vi "HOST_2518.vi"() -> ()   [LabVIEW 2018]
uses:
  <vilib>/userdefined/High Color/nirio_resource_hc.ctl
  <instrlib>/niDCPower/nidcpower.llb/niDCPower Measurement Type.ctl
  <vilib>/FPGAPlugInAG/PXI-7953R/niLvFpga_Open_PXI-7953R.vi
  <vilib>/rvi/interface/common/dynamic/niFpgaDynamicAddResources.vi
  <vilib>/FPGAPlugInAG/Dynamic/niLvFpga_Reset_Dynamic.vi
  <vilib>/FPGAPlugInAG/Dynamic/niLvFpga_Run_Dynamic.vi
  <vilib>/Utility/error.llb/Error Cluster From Error Code.vi
  <vilib>/rvi/errors/niLvFpgaAdjustHostInterfaceError.vi
  <vilib>/FPGAPlugInAG/Dynamic/niLvFpga_Close_Dynamic.vi
  <vilib>/rvi/interface/nirviOpenFPGA/nirviOpenFPGA.xnode
  FPGA Bitfiles/GMAX2518_FPGATarget_Target2518_wpKPnY-EnHw.lvbitx
  <vilib>/rvi/interface/nirviMethod/nirviMethod.xnode
  <vilib>/rvi/interface/nirviReadWriteControl/nirviReadWriteControl.xnode
  <vilib>/rvi/interface/nirviCloseFPGA/nirviCloseFPGA.xnode
  <vilib>/rvi/interface/Simulation/niFpgaSimulationCallBeginRW.vi
  <vilib>/FPGAPlugInAG/Dynamic/niLvFpga_ReadFifo_Dynamic.vi
  <vilib>/rvi/errors/niLvFpgaMergeErrorWithErrorCode.vi
  NiFpgaLv.dll
  <vilib>/FPGAPlugInAG/Dynamic/niLvFpga_StartFifo_Dynamic.vi
  <vilib>/FPGAPlugInAG/Dynamic/niLvFpga_WriteFifo_Dynamic.vi
panel:
  in  "Регистры":u8[](array[numeric])=[35, 5, 0, 100, 1, 0, 1, 0, 0, 0, 0, 0, 55, 16, 0, 0, 0, 69, 0, 6, 0, 160, 15, 0, 0, 0, 0, 0, 0, 0, 0, 0, 0, 0, 0, 0, 0, 0, 0, 0, 0, 0, 0, 0, 0, 0, 0, 0, 0, 0, 0, 0, 0, 0, 0, 0, 0, 0, 0, 0, 0, 0, 0, 0, 0, 0, 0, 0, 0, 0, 0, 0, 0, 0, 0, 0, 0, 0, 0, 0, 0, 0, 0, 52, 16, 0, 0, 6, 8, 2, 4, 0, 1, 33, 35, 2, 184, 100, 9, 50, 1, 160, 240, 255, 255, 255, 255, 255, 255, 255, 255, 255, 255, 255, 255, 2, 12, 80, 0, 25, 5, 76, 82, 65, 20, 3, 192, 96, 196, 71, 2, 12, 176, 3, 15, 48, 224, 240, 81, 72, 4, 192, 128, 196, 71, 62, 8, 1, 196, 255, 75, 164, 161, 64, 14, 65, 252, 31, 129, 12, 152, 0, 28, 28, 1, 8, 0, 0, 133, 2, 60, 64, 0, 18, 5, 224, 0, 196, 72, 1, 0, 3, 3, 48, 124, 20, 202, 68, 0, 0, 0, 0, 0, 0, 0, 0, 0, 0, 0, 0, 0, 0, 128, 0, 27, 33, 192, 83, 98, 60, 11, 16, 119, 196, 221, 13, 227, 143, 42, 0, 0, 0, 0, 0, 81, 0, 138, 162, 40, 40, 10, 138, 190, 31, 28, 1, 1, 0, 0, 40, 40, 40, 40, 232, 0, 0, 0, 0, 0, 0, 0, 0, 0, 0, 0, 0]
  out "Память":i32
  out "Image":T1(plugin-control)
  in  "12":u8=12
  in  "FR":u8=20
  in  "Хватит ждать!":bool
  out "Выкачали из памяти":bool
  out "SEU":u32
  in  "Upd_WR":bool
  out "FIFO_READ":i32
  in  "W(T)/R(F)":bool
  in  "Адрес":u8
  in  "Кол-во":u16=255
  out "НИ":bool
  out "READ":u8[](array[numeric])
  out "Прошили":bool
  in  "SPI":bool
  in  "Обнулить сбои":bool
  in  "Проверка сбоев":bool
  out "世男":bool
  in  "Период опроса, мс":u32=1
  in  "3,3V_LVDS, V":dbl=3.3 caption="voltage level" format="%_6p"
  in  "3,3V_LVDS_curlim":dbl=0.2 caption="current limit" format="%_6p"
  out "3,3V_LVDS_char":dbl(graph)=1.5967060684808935e-06
  in  "VDDPIX, V":dbl=3.6 caption="voltage level" format="%_6p"
  in  "VDDPIX_curlim":dbl=0.3 caption="current limit" format="%_6p"
  out "VDDPIX_char":dbl(graph)=1.5967060684808935e-06
  in  "VG_RSTH, V":dbl=4.1 caption="voltage level" format="%_6p"
  in  "VG_RSTH_curlim":dbl=0.1 caption="current limit" format="%_6p"
  out "VG_RSTH_char":dbl(graph)=1.5967060684808935e-06
  in  "LED, V":dbl=-8.0 caption="voltage level" format="%_6p"
  in  "LED_curlim":dbl=0.1 caption="current limit" format="%_6p"
  out "LED_char":dbl(graph)=1.5967060684808935e-06
  in  "VDD33A, V":dbl=3.3 caption="voltage level" format="%_6p"
  in  "VDD33A_curlim":dbl=0.3 caption="current limit" format="%_6p"
  out "VDD33A_char":dbl(graph)=1.5967060684808935e-06
  in  "VTXH, V":dbl=3.6 caption="voltage level" format="%_6p"
  in  "VDDIO, V":dbl=3.3 caption="voltage level" format="%_6p"
  in  "VDDCL, V":dbl=0.7 caption="voltage level" format="%_6p"
  in  "VDD13, V":dbl=1.3 caption="voltage level" format="%_6p"
  in  "VTXH_curlim":dbl=0.2 caption="current limit" format="%_6p"
  in  "VGRSTL_curlim":dbl=0.1 caption="current limit" format="%_6p"
  in  "VDDIO_curlim":dbl=0.1 caption="current limit" format="%_6p"
  in  "VDDCL_curlim":dbl=0.1 caption="current limit" format="%_6p"
  in  "VTXL_curlim":dbl=0.1 caption="current limit" format="%_6p"
  in  "VDD13_curlim":dbl=1.0 caption="current limit" format="%_6p"
  in  "VGRSTL, V":dbl=-1.3 caption="voltage level" format="%_6p"
  in  "VTXL, V":dbl=-1.3 caption="voltage level" format="%_6p"
  out "VTXH_char":dbl(graph)=-0.007753012065680951
  out "VGRSTL_char":dbl(graph)=6.909391540672134e-05
  out "VDDIO_char":dbl(graph)=9.424895165128459e-05
  out "VDDCL_char":dbl(graph)=-9.950040532110056e-06
  out "VTXL_char":dbl(graph)=9.067752968783287e-05
  out "VDD13_char":dbl(graph)=1.5967060684808935e-06
  in  "VDDPIX_selcur":dbl=0.2 caption="current limit" format="%_6p"
  in  "VDD33A_selcur":dbl=0.2 caption="current limit" format="%_6p"
  in  "VDD13_selcur":dbl=0.75 caption="current limit" format="%_6p"
  in  "VTXL_selcur":dbl=0.09 caption="current limit" format="%_6p"
  out "VDDCL_cur":dbl caption="measurement" format="%_6g"
  out "VTXL_cur":dbl caption="measurement" format="%_6g"
  out "VDD13_cur":dbl caption="measurement" format="%_6g"
  out "VDD33A_cur":dbl caption="measurement" format="%_6g"
  in  "SEL_Time, ms":u32=100
  in  "VG_RSTH_selcur":dbl=0.05 caption="current limit" format="%_6p"
  in  "VTXH_selcur":dbl=0.1 caption="current limit" format="%_6p"
  in  "VGRSTL_selcur":dbl=0.03 caption="current limit" format="%_6p"
  in  "VDDIO_selcur":dbl=0.03 caption="current limit" format="%_6p"
  in  "VDDCL_selcur":dbl=0.02 caption="current limit" format="%_6p"
  out "VDDPIX_cur":dbl caption="measurement" format="%_6g"
  out "VDDIO_cur":dbl caption="measurement" format="%_6g"
  out "VGRSTL_cur":dbl caption="measurement" format="%_6g"
  out "VTXH_cur":dbl caption="measurement" format="%_6g"
  out "VG_RSTH_cur":dbl caption="measurement" format="%_6g"
  out "VDDPIX":u16
  out "VDDPIX":bool
  out "VDD33A":u16
  out "VDD33A":bool
  out "VDD13":u16
  out "VDD13":bool
  out "VTXL":u16
  out "VTXL":bool
  in  "3":refnum<k15>="PXI1Slot5" caption="1"
  in  "MOVIE":bool
  in  "FRAME!":bool
  out "SEL":bool
  in  "SIM_SEL":bool
  out "VG_RSTH":u16
  out "VDDCL":u16
  out "VTXH":u16
  out "VDDIO":u16
  out "VGRSTL":u16
  out "VG_RSTH":bool
  out "VDDCL":bool
  out "VTXH":bool
  out "VDDIO":bool
  out "VGRSTL":bool
  in  "Стоп":bool
  in  "Питание":bool
  in  "LED":bool caption="output enabled"
  in  "0":refnum<k15>="PXI1Slot2" caption="1"
  in  "1":refnum<k15>="PXI1Slot3"
  in  "2":refnum<k15>="PXI1Slot4" caption="1"
  in  "resource name 2":T2="PXI1Slot6"
  in  "SEU":path=path "C:/LabView_PRJ/GMAX2518/SEU"
  in  "SEL":path=path "C:/LabView_PRJ/GMAX2518/SEL"
  out "Номер образца":string="1"
  # "0-163 тест (35)"
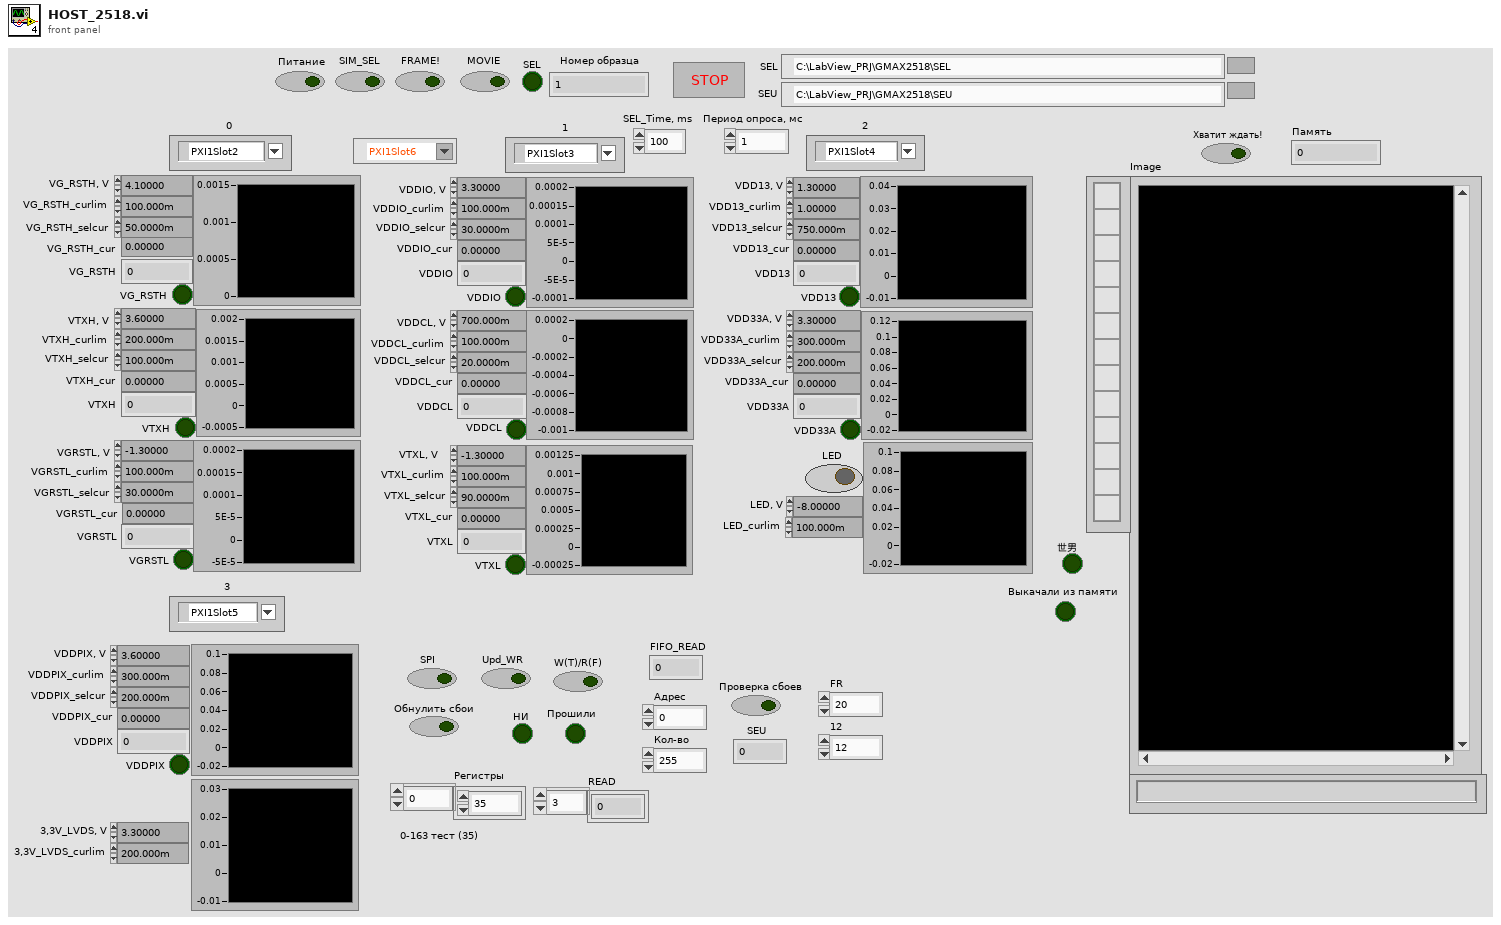
[diagram p1: front panel]
types:
  T1 = typedef "IMAQ Image.ctl" = refnum<image>
  T2 = typedef "nirio_resource_hc.ctl" = tag
  T3 = typedef "Image Type" = u32
  T4 = enum16{"open", "replace", "create", "open or create", "replace or create", "replace or create with confirmation"}
  T5 = typedef "niDCPower Measurement Type.ctl" = i32
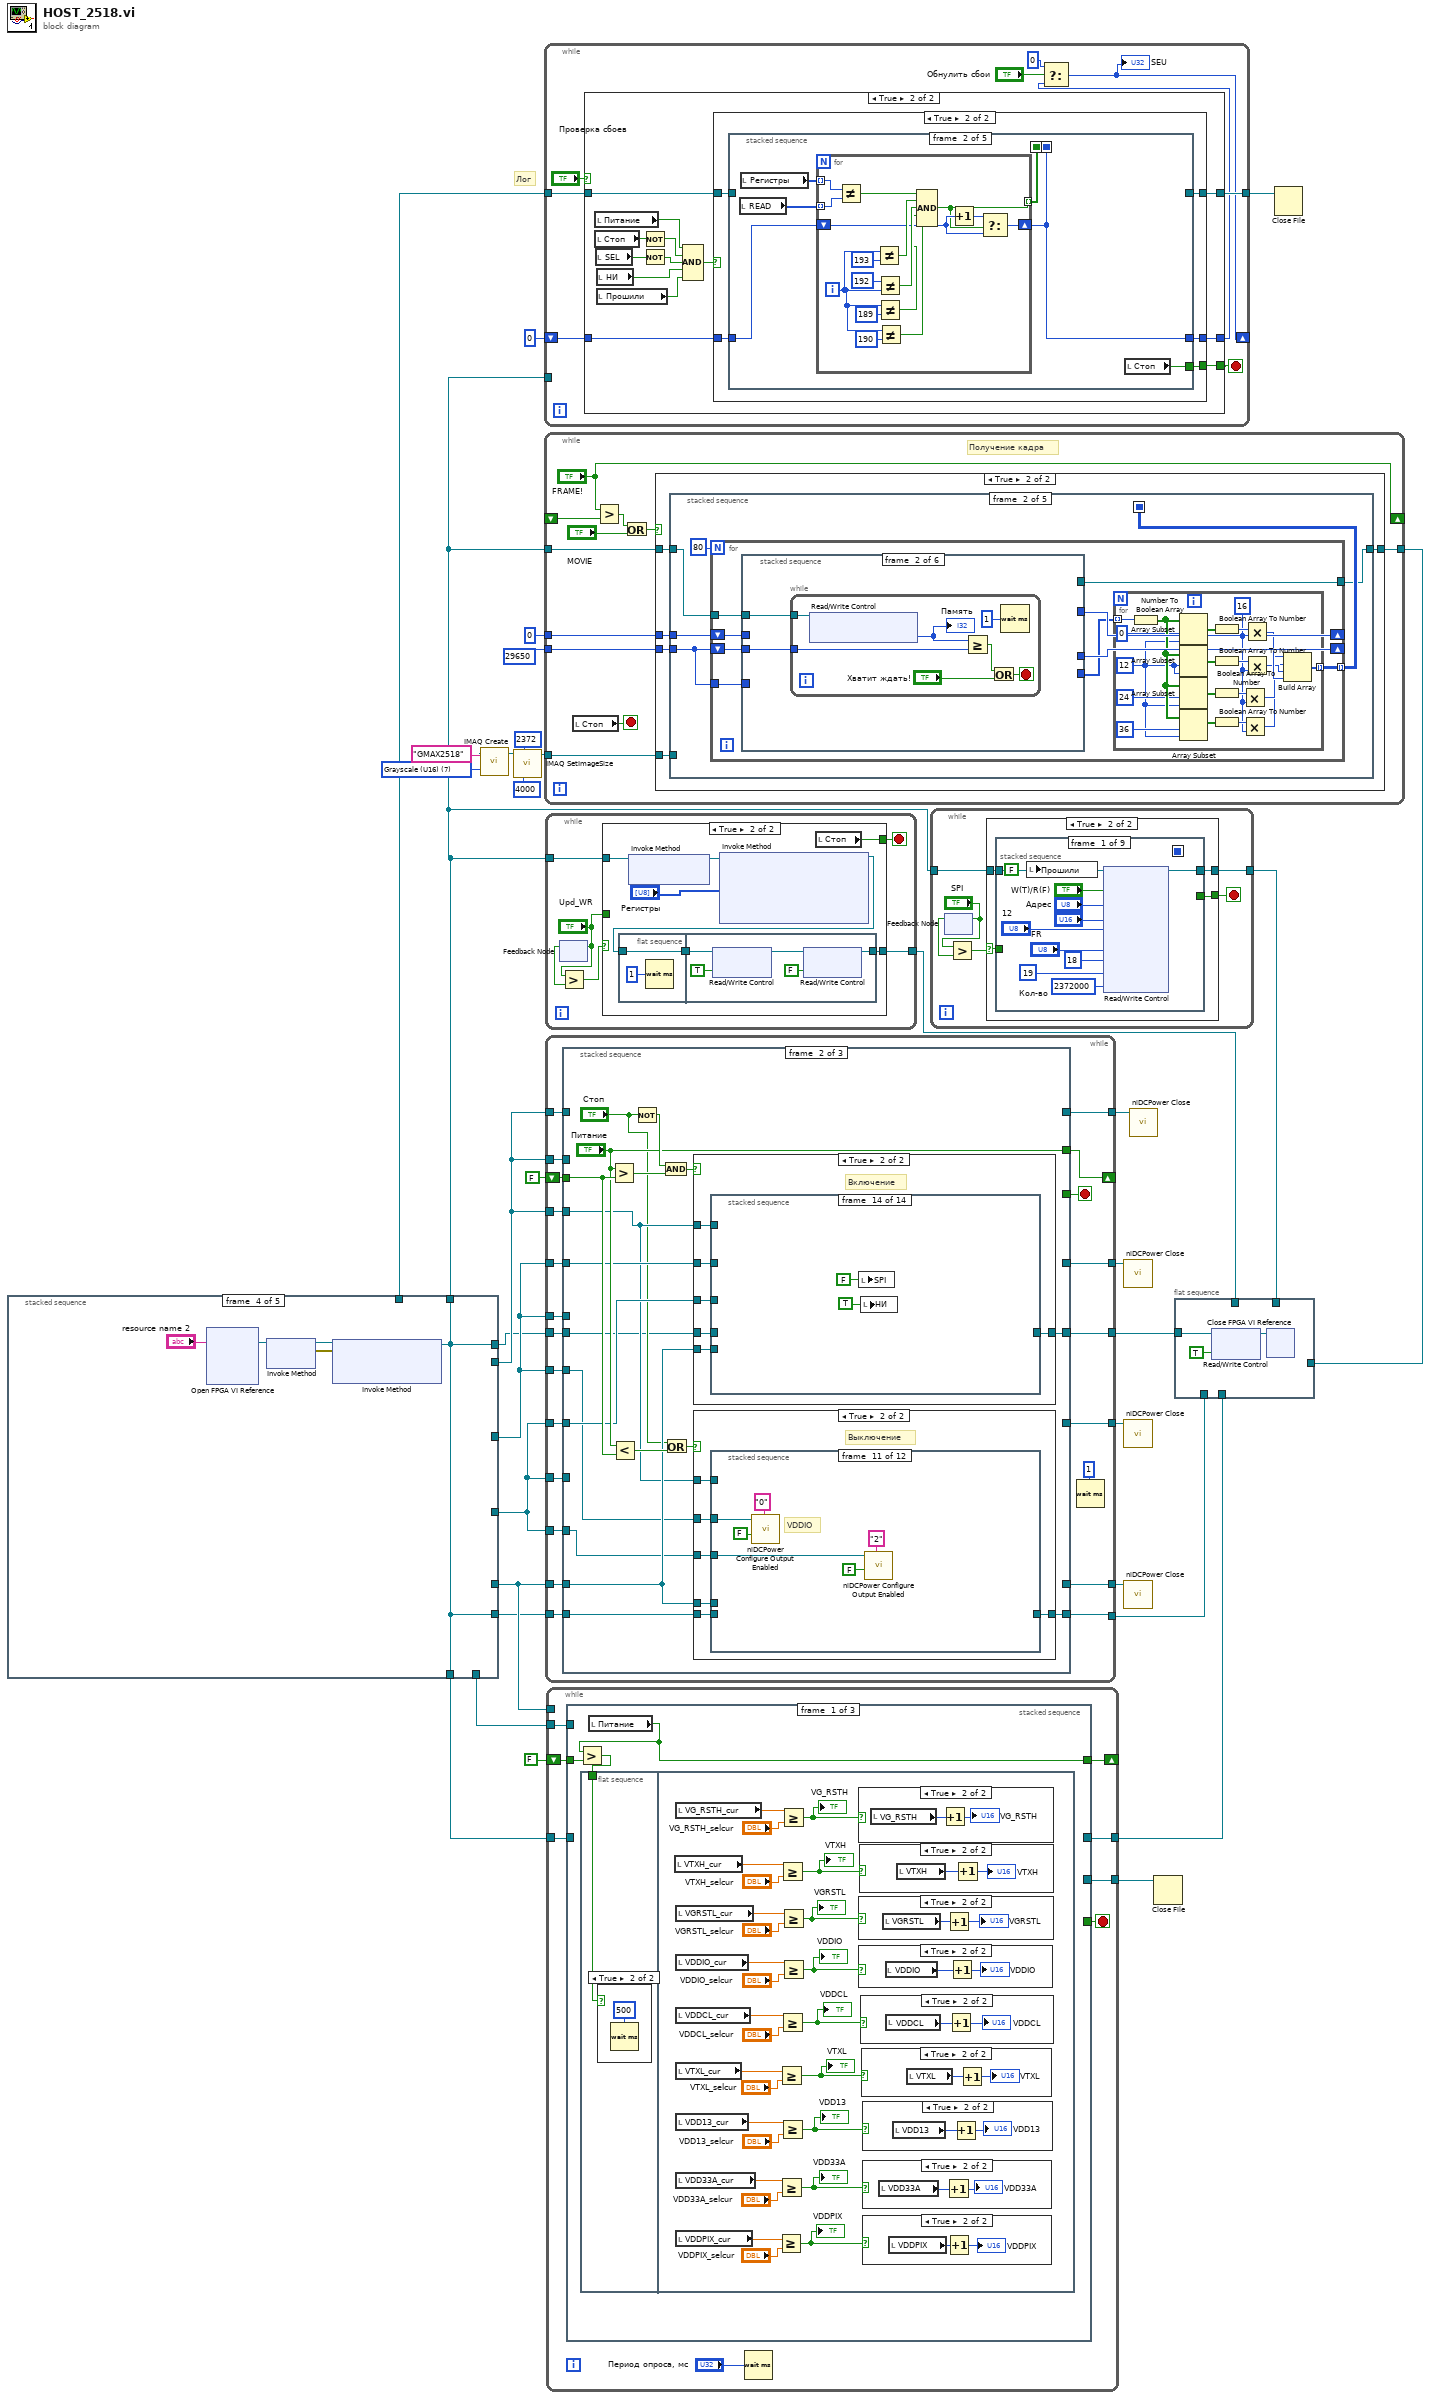
[diagram p0: block diagram]
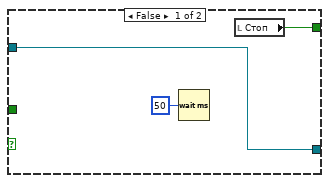
[diagram p2: hidden frame]
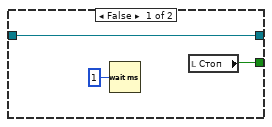
[diagram p3: hidden frame]
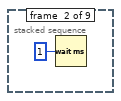
[diagram p4: hidden frame]
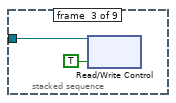
[diagram p5: hidden frame]
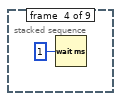
[diagram p6: hidden frame]
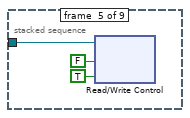
[diagram p7: hidden frame]
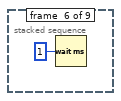
[diagram p8: hidden frame]
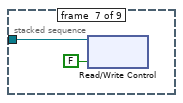
[diagram p9: hidden frame]
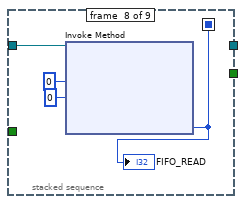
[diagram p10: hidden frame]
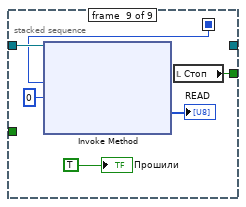
[diagram p11: hidden frame]
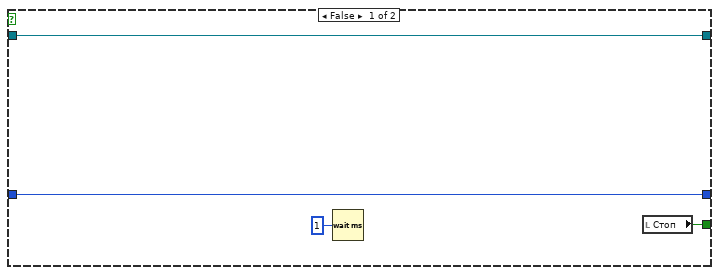
[diagram p12: hidden frame]
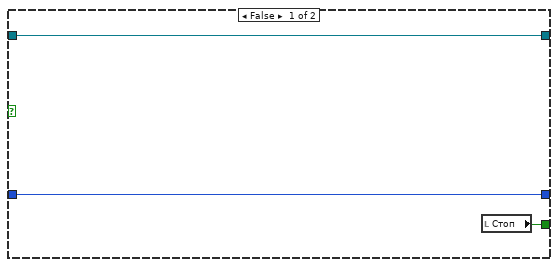
[diagram p13: hidden frame]
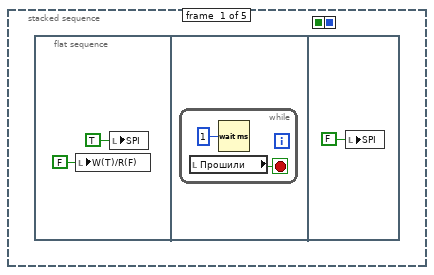
[diagram p14: hidden frame]
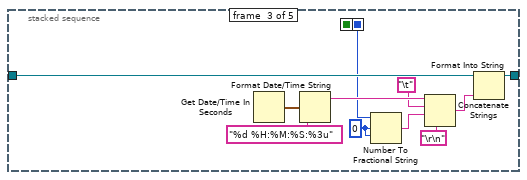
[diagram p15: hidden frame]
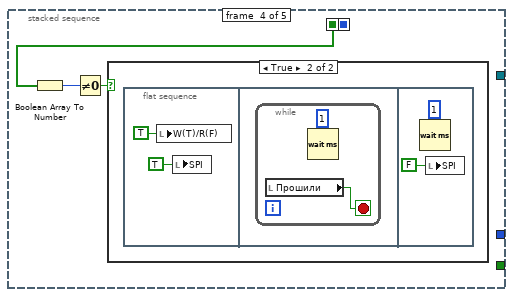
[diagram p16: hidden frame]
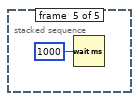
[diagram p18: hidden frame]
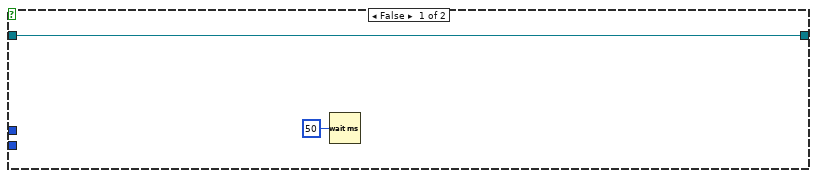
[diagram p19: hidden frame]
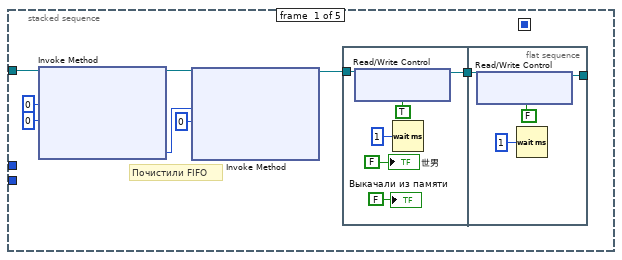
[diagram p20: hidden frame]
diagram:
  w20 = T3 7 items=["Grayscale (U8)", "Grayscale (I16)", "Grayscale (SGL)", "Complex (CSG)", "RGB (U32)", "HSL (U32)", "RGB (U64)", "Grayscale (U16)"] ("Image Type")
  # "Лог"
  n1 = stacked-sequence {
    tunnel: [_ _ _ _ w118] -> w26
    tunnel: [_ _ _ _ w111] -> w21
    tunnel: [_ _ _ _ w122] -> w27
    tunnel: [_ _ _ w106 _] -> w13
    tunnel: [_ _ _ w106 _] -> w30
    tunnel: [_ w45 _ _ _] -> w31
    tunnel: [_ _ _ w106 _] -> w12
    tunnel: [_ _ _ _ w112] -> w28
    tunnel: [_ _ w75 _ _] -> w1
    tunnel: [_ _ _ w106 _] -> w10
    frame #0 {
      w35 = FALSE ("Стоп")
      w34 = FALSE ("Стоп")
      w36 = u16 0 ("ADC")
      # "Обнуление"
      n2 = call "Begin.vi"() -> ("Номер образца 2"=→"Номер образца":string)  [unwired: 11 in]
      n3 = local write "VTXH"(w35) -> ()
      n4 = local write "SIM_SEL"(w35) -> ()
      n5 = local write "SEL"(w35) -> ()
      n6 = local write "VTXL"(w35) -> ()
      n7 = local write "VDD13"(w35) -> ()
      n8 = local write "VDD33A"(w35) -> ()
      n9 = local write "VDDPIX"(w35) -> ()
      n10 = local write "VTXH"(w36) -> ()
      n11 = local write "VDDCL"(w36) -> ()
      n12 = local write "VG_RSTH"(w36) -> ()
      n13 = local write "VDDIO"(w36) -> ()
      n14 = local write "VGRSTL"(w36) -> ()
      n15 = local write "VTXL"(w36) -> ()
      n16 = local write "VDD13"(w36) -> ()
      n17 = local write "VDD33A"(w36) -> ()
      n18 = local write "VDDPIX"(w36) -> ()
      n19 = local write "Стоп"(w34) -> ()
      n20 = local write "Питание"(w34) -> ()
      n21 = local write "FRAME!"(w34) -> ()
      n22 = local write "MOVIE"(w34) -> ()
      n23 = local write "LED"(w34) -> ()
      n24 = local write "VG_RSTH"(w34) -> ()
      n25 = local write "VDDCL"(w34) -> ()
      n26 = local write "VGRSTL"(w34) -> ()
      n27 = local write "VDDIO"(w34) -> ()
      n28 = local write "Выкачали из памяти"(w34) -> ()
    }
    frame #1 {
      w40 = "\t"
      # "Лог по токам"
      n29 = local read "Номер образца"() -> (w67:string)
      n30 = Build Path(base path="SEL", name or relative path=w67) -> (appended path=w64:path)
      n31 = Get Date/Time In Seconds() -> (seconds since 1Jan1904=w61:timestamp)
      n32 = call <vilib>:"Check if File or Folder Exists.vi"("path"=w64) -> ("file or folder exists?"=w65:bool, "dup path"=w66:path)  [unwired: 8 in, 1 out]
      n33 = Format Date/Time String(time format string (%c)="%d %H.%M.%S", seconds (now)=w61) -> (date/time string=w59:string)  [unwired: 1 in]
      n34 = case shown="False" w65 {
        tunnel: w66 -> [w73 w74]
        tunnel: [w72 w74] -> w39
        frame False {
          n35 = Create Folder(path (use dialog)=w73) -> (created path=w72:path)  [unwired: 2 in, 2 out]
        }
        frame True {
        }
      }
      n36 = Concatenate Strings(w59, ".xls" ("string")) -> (w58:string)
      n37 = Build Path(base path=w39, name or relative path=w58) -> (appended path=w60:path)
      n38 = Open/Create/Replace File(file path (use dialog)=w60, operation (0:open)=T4."open or create", access (0:read/write)=enum16{"read/write", "read-only", "write-only"}."read/write") -> (refnum out=w62:refnum<file>)  [unwired: 3 in, 2 out]
      n39 = case shown="True" TRUE {
        tunnel: w62 -> [w68 w71]
        tunnel: [w68 w69] -> w57
        frame False {
        }
        frame True {
          n40 = Set File Position(refnum=w71, from (0:start)=enum16{"start", "end", "current"}."end") -> (refnum out=w69:refnum<file>)  [unwired: 2 in, 1 out]
        }
      }
      n41 = Format Into String(initial string=w57, "Time" ("input 1"), w40, "VG_RSTH_cur", w40, "VTXH_cur", w40, "VGRSTL_cur", w40, "VDDIO_cur", w40, "VDDCL_cur", w40, "VTXL_cur", w40, "VDD13_cur", w40, "VDD33A_cur", w40, "VDDPIX_cur", w40, "\r\n") -> (resulting string=w45:refnum<file>)  [unwired: 2 in, 1 out]
    }
    frame #2 {
      w78 = "\t"
      # "Лог по сбоям"
      n42 = local read "Номер образца"() -> (w82:string)
      n43 = Build Path(base path="SEU", name or relative path=w82) -> (appended path=w96:path)
      n44 = Get Date/Time In Seconds() -> (seconds since 1Jan1904=w94:timestamp)
      n45 = call <vilib>:"Check if File or Folder Exists.vi"("path"=w96) -> ("file or folder exists?"=w97:bool, "dup path"=w98:path)  [unwired: 8 in, 1 out]
      n46 = Format Date/Time String(time format string (%c)="%d %H.%M.%S", seconds (now)=w94) -> (date/time string=w92:string)  [unwired: 1 in]
      n47 = case shown="False" w97 {
        tunnel: w98 -> [w104 w105]
        tunnel: [w103 w105] -> w83
        frame False {
          n48 = Create Folder(path (use dialog)=w104) -> (created path=w103:path)  [unwired: 2 in, 2 out]
        }
        frame True {
        }
      }
      n49 = Concatenate Strings(w92, ".xls" ("string")) -> (w91:string)
      n50 = Build Path(base path=w83, name or relative path=w91) -> (appended path=w93:path)
      n51 = Open/Create/Replace File(file path (use dialog)=w93, operation (0:open)=T4."open or create", access (0:read/write)=enum16{"read/write", "read-only", "write-only"}."read/write") -> (refnum out=w95:refnum<file>)  [unwired: 3 in, 2 out]
      n52 = case shown="True" TRUE {
        tunnel: w95 -> [w99 w102]
        tunnel: [w99 w100] -> w90
        frame False {
        }
        frame True {
          n53 = Set File Position(refnum=w102, from (0:start)=enum16{"start", "end", "current"}."end") -> (refnum out=w100:refnum<file>)  [unwired: 2 in, 1 out]
        }
      }
      n54 = Format Into String(initial string=w90, "Time" ("input 1"), w78, "Регистр №" ("input 3"), w78, "Содержание" ("input 4"), w78, "Кол-во сбоев" ("input 7"), "\r\n") -> (resulting string=w75:refnum<file>)  [unwired: 2 in, 1 out]
    }
    frame #3 {
      n55 = xnode "Open FPGA VI Reference"("resource name"="resource name 2") -> ("FPGA VI Reference Out"=w107:refnum<k20>)  [unwired: 1 in, 1 out]
      n56 = xnode "Invoke Method"("FPGA VI Reference In"=w107) -> ("FPGA VI Reference Out"=w110:refnum<k20>, "error out"=w109:errorcluster)  [unwired: 1 in]
      n57 = xnode "Invoke Method"("FPGA VI Reference In"=w110, "error in"=w109) -> ("FPGA VI Reference Out"=w106:refnum<k20>)  [unwired: 1 in, 1 out]
    }
    frame #4 {
      n58 = call <instrlib>:"niDCPower Initialize.vi"("resource name"="2") -> ("error out"=w128:errorcluster, "instrument handle out"=w125:refnum<k15>)  [unwired: 3 in, 6 out]
      n59 = call <instrlib>:"niDCPower Initialize.vi"("resource name"="1") -> ("error out"=w126:errorcluster, "instrument handle out"=w123:refnum<k15>)  [unwired: 3 in, 6 out]
      n60 = call <instrlib>:"niDCPower Initialize.vi"("resource name"="3") -> ("error out"=w116:errorcluster, "instrument handle out"=w117:refnum<k15>)  [unwired: 3 in, 6 out]
      n61 = call <instrlib>:"niDCPower Initialize.vi"("resource name"="0") -> ("error out"=w127:errorcluster, "instrument handle out"=w124:refnum<k15>)  [unwired: 3 in, 6 out]
      n62 = call <instrlib>:"niDCPower Configure Voltage Level.vi"("error in (no error)"=w128, "voltage level"=0.0, "channel name"="0,1,2", "instrument handle"=w125) -> ("instrument handle out"=w118:refnum<k15>)  [unwired: 6 in, 1 out]
      n63 = call <instrlib>:"niDCPower Configure Voltage Level.vi"("error in (no error)"=w126, "voltage level"=0.0, "channel name"="0,1,2", "instrument handle"=w123) -> ("instrument handle out"=w122:refnum<k15>)  [unwired: 6 in, 1 out]
      n64 = call <instrlib>:"niDCPower Configure Voltage Level.vi"("error in (no error)"=w116, "voltage level"=0.0, "channel name"="0,1", "instrument handle"=w117) -> ("instrument handle out"=w112:refnum<k15>)  [unwired: 6 in, 1 out]
      n65 = call <instrlib>:"niDCPower Configure Voltage Level.vi"("error in (no error)"=w127, "voltage level"=0.0, "channel name"="0,1,2", "instrument handle"=w124) -> ("instrument handle out"=w111:refnum<k15>)  [unwired: 6 in, 1 out]
    }
  }
  n66 = call "IMAQ Create"("Image Name"="GMAX2518", "Image Type"=w20) -> ("New Image"=w3:T1)  [unwired: 3 in, 1 out]
  n67 = call "IMAQ SetImageSize"("Y Resolution"=4000, "X Resolution"=2372, "Image"=w3) -> ("Image Out"=w6:T1)  [unwired: 2 in, 1 out]
  n68 = while {
    tunnel: w1 -> [w143]
    tunnel: [w142] -> w14
    shift-right: [w135] -> _
    shift-left: u32 0 -> [w139]
    tunnel: w13 -> [_]
    stop <- w140 stop-if-true
    n69 = case shown="True" "Проверка сбоев" {
      tunnel: [w145 w153] -> w140
      tunnel: w143 -> [w146 w154]
      tunnel: [w146 w150] -> w142
      tunnel: w139 -> [w144 w152]
      tunnel: [w144 w151] -> w138
      frame False {
        n70 = Wait (ms)(milliseconds to wait=u32 1) -> ()  [unwired: 1 out]
        n71 = local read "Стоп"() -> (w145:bool)
      }
      frame True {
        n72 = local read "Питание"() -> (w159:bool)
        n73 = local read "Стоп"() -> (w160:bool)
        n74 = local read "SEL"() -> (w149:bool)
        n75 = local read "НИ"() -> (w156:bool)
        n76 = local read "Прошили"() -> (w148:bool)
        n77 = Not(x=w160) -> (.not. x?=w158:bool)
        n78 = Not(x=w149) -> (.not. x?=w157:bool)
        n79 = Compound Arithmetic op=AND(w159, w158, w157, w156, w148) -> (w155:bool)
        n80 = case shown="True" w155 {
          tunnel: w154 -> [w161 w168]
          tunnel: [w163 w167] -> w153
          tunnel: w152 -> [w162 w166]
          tunnel: [w162 w165] -> w151
          tunnel: [w161 w164] -> w150
          frame False {
            n81 = local read "Стоп"() -> (w163:bool)
          }
          frame True {
            n82 = stacked-sequence {
              seq-local: [_ w175 _ _ _] -> [_ _ w200 _ _]
              seq-local: [_ w174 _ _ _] -> [_ _ _ w207 _]
              tunnel: w168 -> [_ _ w205 _ _]
              tunnel: [_ w179 _ _ _] -> w167
              tunnel: w166 -> [_ w176 _ _ _]
              tunnel: [_ w175 _ _ _] -> w165
              tunnel: [_ _ w196 _ _] -> w164
              frame #0 {
                n83 = flat-sequence {
                  frame #0 {
                    n84 = local write "W(T)/R(F)"(FALSE ("W(T)/R(F)")) -> ()
                    n85 = local write "SPI"(TRUE ("SPI")) -> ()
                  }
                  frame #1 {
                    n86 = while {
                      stop <- w172 stop-if-true
                      n87 = local read "Прошили"() -> (w172:bool)
                      n88 = Wait (ms)(milliseconds to wait=u32 1) -> ()  [unwired: 1 out]
                    }
                  }
                  frame #2 {
                    n89 = local write "SPI"(FALSE ("SPI")) -> ()
                  }
                }
              }
              frame #1 {
                n90 = local read "READ"() -> (w178:u8[])
                n91 = local read "Регистры"() -> (w177:u8[])
                n92 = for {
                  tunnel: w178 -> [w189] mode=indexing
                  tunnel: w177 -> [w195] mode=indexing
                  shift-right: [w186] -> w175
                  shift-left: w176 -> [w187]
                  tunnel: [w185] -> w174 mode=indexing
                  i -> [w184]
                  n93 = Not Equal?(x=w195, y=w189) -> (x != y?=w192:bool)
                  n94 = Not Equal?(x=w184, y=193) -> (x != y?=w191:bool)
                  n95 = Not Equal?(x=192, y=w184) -> (x != y?=w190:bool)
                  n96 = Not Equal?(x=w184, y=189) -> (x != y?=w183:bool)
                  n97 = Not Equal?(x=w184, y=190) -> (x != y?=w182:bool)
                  n98 = Compound Arithmetic op=AND(w192, w191, w190, w183, w182) -> (w185:bool)
                  n99 = Increment(x=w187) -> (x+1=w188:u32)
                  n100 = Select(t=w188, s=w185, f=w187) -> (s? t:f=w186:u32)
                }
                n101 = local read "Стоп"() -> (w179:bool)
              }
              frame #2 {
                w199 = i16 0 ("width (-)")
                n102 = Get Date/Time In Seconds() -> (seconds since 1Jan1904=w204:timestamp)
                n103 = Format Date/Time String(time format string (%c)="%d %H:%M:%S:%3u", seconds (now)=w204) -> (date/time string=w202:string)  [unwired: 1 in]
                n104 = Number To Fractional String(number=w200, width (-)=w199, precision (6)=w199) -> (F-format string=w198:string)  [unwired: 1 in]
                n105 = Concatenate Strings(w202, "\t", w198, "\r\n") -> (w206:string)
                n106 = Format Into String(initial string=w205, w206) -> (resulting string=w196:refnum<file>)  [unwired: 2 in, 1 out]
              }
              frame #3 {
                n107 = Boolean Array To Number(Boolean array=w207) -> (number=w209:u32)
                n108 = Not Equal To 0?(x=w209) -> (x != 0?=w208:bool)
                n109 = case shown="True" w208 {
                  frame False {
                  }
                  frame True {
                    n110 = flat-sequence {
                      frame #0 {
                        n111 = local write "W(T)/R(F)"(TRUE ("W(T)/R(F)")) -> ()
                        n112 = local write "SPI"(TRUE ("SPI")) -> ()
                      }
                      frame #1 {
                        n113 = while {
                          stop <- w213 stop-if-true
                          n114 = local read "Прошили"() -> (w213:bool)
                          n115 = Wait (ms)(milliseconds to wait=u32 1) -> ()  [unwired: 1 out]
                        }
                      }
                      frame #2 {
                        n116 = Wait (ms)(milliseconds to wait=u32 1) -> ()  [unwired: 1 out]
                        n117 = local write "SPI"(FALSE ("SPI")) -> ()
                      }
                    }
                  }
                }
              }
              frame #4 {
                n118 = Wait (ms)(milliseconds to wait=u32 1000) -> ()  [unwired: 1 out]
              }
            }
          }
        }
      }
    }
    n119 = Select(t=u32 0, s="Обнулить сбои", f=w138) -> (s? t:f=w135:u32)
    "SEU" <- w135
  }
  n120 = while {
    tunnel: w13 -> [w224]
    shift-right: ["FRAME!"] -> _
    shift-left: _ -> [w227]
    tunnel: u32 0 -> [w223]
    tunnel: u32 29650 ("163840") -> [w222]
    tunnel: w6 -> [w218]
    tunnel: [w217] -> w2
    stop <- w221 stop-if-true
    # "Получение кадра"
    n121 = local read "Стоп"() -> (w221:bool)
    n122 = Greater?(x="FRAME!", y=w227) -> (0:w226:bool)
    n123 = Or(x=w226, y="MOVIE") -> (x .or. y?=w225:bool)
    n124 = case shown="True" w225 {
      tunnel: w224 -> [w228 w234]
      tunnel: w223 -> [_ w233]
      tunnel: w222 -> [_ w232]
      tunnel: w218 -> [_ w231]
      tunnel: [w228 w230] -> w217
      frame False {
        n125 = Wait (ms)(milliseconds to wait=u32 50) -> ()  [unwired: 1 out]
      }
      frame True {
        n126 = stacked-sequence {
          seq-local: [_ w254 _ _ _] -> [_ _ _ w322 _]
          tunnel: w234 -> [w238 w255 _ _ w336]
          tunnel: w233 -> [_ w257 _ _ _]
          tunnel: w232 -> [_ w256 _ _ _]
          tunnel: w231 -> [_ _ _ w329 _]
          tunnel: [_ w253 _ _ _] -> w230
          frame #0 {
            # "Почистили FIFO"
            n127 = xnode "Invoke Method"("FPGA VI Reference In"=w238, "Number of Elements"=u32 0, "Timeout (ms)"=0) -> ("FPGA VI Reference Out"=w237:refnum<k20>, "Elements Remaining"=w239:u32)  [unwired: 1 in, 2 out]
            n128 = xnode "Invoke Method"("FPGA VI Reference In"=w237, "Number of Elements"=w239, "Timeout (ms)"=0) -> ("FPGA VI Reference Out"=w236:refnum<k20>)  [unwired: 1 in, 3 out]
            n129 = flat-sequence {
              tunnel: w236 -> [w248]
              tunnel: [w244] -> w235
              tunnel: [w250] -> _
              tunnel: w235 -> [w249]
              frame #0 {
                n130 = xnode "Read/Write Control"("FPGA VI Reference In"=w248, "Кадр в память"=TRUE ("EXPOSURE")) -> ("FPGA VI Reference Out"=w244:refnum<k20>)  [unwired: 1 in, 1 out]
                n131 = Wait (ms)(milliseconds to wait=u32 1) -> ()  [unwired: 1 out]
                "世男" <- FALSE
                "Выкачали из памяти" <- FALSE ("Выкачали из памяти")
              }
              frame #1 {
                n132 = xnode "Read/Write Control"("FPGA VI Reference In"=w249, "Кадр в память"=FALSE) -> ("FPGA VI Reference Out"=w250:refnum<k20>)  [unwired: 1 in, 1 out]
                n133 = Wait (ms)(milliseconds to wait=u32 1) -> ()  [unwired: 1 out]
              }
            }
          }
          frame #1 {
            n134 = for {
              N: 80 -> [_]
              tunnel: w255 -> [w267]
              shift-right: [w264] -> _
              shift-left: w257 -> [w266]
              shift-right: [w263] -> _
              shift-left: w256 -> [w265]
              tunnel: w256 -> [w262]
              tunnel: [w260] -> w254 mode=indexing
              tunnel: [w259] -> w253
              n135 = stacked-sequence {
                tunnel: w267 -> [w293 w294 w303 w305 w307 w313]
                tunnel: w266 -> [w292 _ _ _ _ _]
                tunnel: w265 -> [w291 w295 _ _ _ _]
                tunnel: [w290 _ _ _ _ _] -> w264
                tunnel: [w289 _ _ _ _ _] -> w263
                tunnel: [_ _ _ _ _ w315] -> w261
                tunnel: [_ _ _ _ _ w314] -> w259
                tunnel: w262 -> [w288 _ _ _ _ _]
                frame #0 {
                  n136 = xnode "Read/Write Control"("FPGA VI Reference In"=w293, "Нач_адр"=w292, "Кон_адр"=w291) -> ()  [unwired: 1 in, 2 out]
                  n137 = Add(x=w292, y=w288) -> (x+y=w290:u32)
                  n138 = Add(x=w288, y=w291) -> (x+y=w289:u32)
                }
                frame #1 {
                  n139 = while {
                    tunnel: w295 -> [w300]
                    tunnel: w294 -> [w298]
                    stop <- w299 stop-if-true
                    n140 = xnode "Read/Write Control"("FPGA VI Reference In"=w298) -> ("Записали адресов"=w296:u32)  [unwired: 1 in, 2 out]
                    "Память" <- w296
                    n141 = Greater Or Equal?(x=w296, y=w300) -> (x >= y?=w302:bool)
                    n142 = Or(x=w302, y="Хватит ждать!") -> (x .or. y?=w299:bool)
                    n143 = Wait (ms)(milliseconds to wait=u32 1) -> ()  [unwired: 1 out]
                  }
                }
                frame #2 {
                  n144 = xnode "Read/Write Control"("FPGA VI Reference In"=w303, "Кадр на ПК"=TRUE ("HOST")) -> ()  [unwired: 1 in, 2 out]
                }
                frame #3 {
                  n145 = xnode "Read/Write Control"("FPGA VI Reference In"=w305, "Кадр на ПК"=FALSE ("HOST")) -> ()  [unwired: 1 in, 2 out]
                }
                frame #4 {
                  n146 = while {
                    tunnel: w307 -> [w309]
                    stop <- w310 stop-if-true
                    # "Записан FIFO?"
                    n147 = local read "Хватит ждать!"() -> (w308:bool)
                    n148 = xnode "Read/Write Control"("FPGA VI Reference In"=w309) -> ("Записали FIFO"=w311:bool)  [unwired: 1 in, 2 out]
                    n149 = Or(x=w311, y=w308) -> (x .or. y?=w310:bool)
                    n150 = Wait (ms)(milliseconds to wait=u32 1) -> ()  [unwired: 1 out]
                  }
                }
                frame #5 {
                  n151 = xnode "Invoke Method"("FPGA VI Reference In"=w313, "Number of Elements"=u32 0, "Timeout (ms)"=0) -> ("FPGA VI Reference Out"=w319:refnum<k20>, "Elements Remaining"=w320:u32)  [unwired: 1 in, 2 out]
                  n152 = xnode "Invoke Method"("FPGA VI Reference In"=w319, "Number of Elements"=w320, "Timeout (ms)"=0) -> ("FPGA VI Reference Out"=w314:refnum<k20>, "Data"=w315:u64[])  [unwired: 1 in, 2 out]
                }
              }
              n153 = for {
                tunnel: w261 -> [w287] mode=indexing
                tunnel: [w281] -> w260 mode=indexing
                w272 = u16 16
                w282 = 12 ("index")
                n154 = Number To Boolean Array(number=w287) -> (Boolean array=w286:bool[])
                n155 = Array Subset(array=w286, index=0, length=w282) -> (w280:bool[])
                n156 = Array Subset(array=w286, index=w282, length=w282) -> (w279:bool[])
                n157 = Array Subset(array=w286, index=24, length=w282) -> (w278:bool[])
                n158 = Array Subset(array=w286, index=36, length=w282) -> (w277:bool[])
                n159 = Boolean Array To Number(Boolean array=w280) -> (number=w276:u16)
                n160 = Boolean Array To Number(Boolean array=w279) -> (number=w275:u16)
                n161 = Boolean Array To Number(Boolean array=w278) -> (number=w274:u16)
                n162 = Boolean Array To Number(Boolean array=w277) -> (number=w273:u16)
                n163 = Multiply(x=w274, y=w272) -> (x*y=w269:u16)
                n164 = Multiply(x=w273, y=w272) -> (x*y=w268:u16)
                n165 = Multiply(x=w276, y=w272) -> (x*y=w271:u16)
                n166 = Multiply(x=w275, y=w272) -> (x*y=w270:u16)
                n167 = Build Array(w268, w269, w270, w271) -> (w281:u16[])
              }
            }
          }
          frame #2 {
            n168 = local write "Выкачали из памяти"(TRUE ("Выкачали из памяти")) -> ()
          }
          frame #3 {
            # "Парсинг"
            n169 = Reshape Array(w322, 9488000 ("dimension size")) -> (w327:u16[])
            n170 = for {
              N: 4000 ("6032") -> [_]
              shift-right: [w334] -> _
              shift-left: 0 ("index") -> [w333]
              tunnel: [w332] -> w326 mode=indexing
              tunnel: w327 -> [w330]
              w331 = 2372 ("3964")
              n171 = Array Subset(array=w330, index=w333, length=w331) -> (w332:u16[])
              n172 = Add(x=w331, y=w333) -> (x+y=w334:i32)
            }
            n173 = call "IMAQ ArrayToImage"("Image Pixels (U16)"=w326, "Image"=w329) -> ("Image Out"=→"Image":T1)  [unwired: 8 in, 1 out]
          }
          frame #4 {
            n174 = local read "Хватит ждать!"() -> (w335:bool)
            n175 = local write "世男"(TRUE ("世男")) -> ()
            n176 = xnode "Read/Write Control"("FPGA VI Reference In"=w336, "Хватит"=w335) -> ()  [unwired: 1 in, 2 out]
          }
        }
      }
    }
  }
  n177 = while {
    tunnel: w13 -> [w340]
    tunnel: [w338] -> w7
    stop <- w342 stop-if-true
    n178 = feedback-in #1("Upd_WR") -> ()
    n179 = feedback #1() -> (w343:bool)  [unwired: 1 in]
    n180 = Greater?(x="Upd_WR", y=w343) -> (0:w341:bool)
    n181 = case shown="True" w341 {
      tunnel: [w345 w353] -> w342
      tunnel: w340 -> [w344 w350]
      tunnel: "Upd_WR" -> [_ _]
      tunnel: [w344 w348] -> w338
      frame False {
        n182 = Wait (ms)(milliseconds to wait=u32 50) -> ()  [unwired: 1 out]
        n183 = local read "Стоп"() -> (w345:bool)
      }
      frame True {
        n184 = flat-sequence {
          tunnel: w352 -> [w355]
          tunnel: [w355] -> w349
          tunnel: w349 -> [w360]
          tunnel: [w356] -> w348
          frame #0 {
            n185 = Wait (ms)(milliseconds to wait=u32 1) -> ()  [unwired: 1 out]
          }
          frame #1 {
            n186 = xnode "Read/Write Control"("FPGA VI Reference In"=w360, "Upd_WR"=TRUE) -> ("FPGA VI Reference Out"=w359:refnum<k20>)  [unwired: 1 in, 1 out]
            n187 = xnode "Read/Write Control"("FPGA VI Reference In"=w359, "Upd_WR"=FALSE) -> ("FPGA VI Reference Out"=w356:refnum<k20>)  [unwired: 1 in, 1 out]
          }
        }
        n188 = xnode "Invoke Method"("FPGA VI Reference In"=w350) -> ("FPGA VI Reference Out"=w351:refnum<k20>)  [unwired: 1 in, 1 out]
        n189 = xnode "Invoke Method"("FPGA VI Reference In"=w351, "Data"="Регистры") -> ("FPGA VI Reference Out"=w352:refnum<k20>)  [unwired: 2 in, 2 out]
        n190 = local read "Стоп"() -> (w353:bool)
      }
    }
  }
  n191 = while {
    shift-right: [w381] -> _
    shift-left: FALSE -> [w382]
    tunnel: w21 -> [w380]
    tunnel: w27 -> [w374]
    tunnel: w26 -> [w371]
    tunnel: w28 -> [w379]
    tunnel: w21 -> [w376]
    tunnel: w21 -> [w375]
    tunnel: w27 -> [w373]
    tunnel: w27 -> [w372]
    tunnel: w26 -> [w370]
    tunnel: w26 -> [w369]
    tunnel: [w368] -> w25
    tunnel: [w367] -> w24
    tunnel: [w366] -> w23
    tunnel: [w365] -> w22
    tunnel: w12 -> [w364]
    tunnel: [w363] -> w11
    tunnel: w10 -> [w362]
    tunnel: [w361] -> w9
    stop <- w378 stop-if-true
    n192 = stacked-sequence {
      tunnel: w382 -> [_ w502 _]
      tunnel: [_ "Питание" _] -> w381
      tunnel: w380 -> [w394 _ w587]
      tunnel: w379 -> [w383 w493 w584]
      tunnel: [_ _ w588] -> w378
      tunnel: w376 -> [w393 _ _]
      tunnel: w375 -> [w392 w490 _]
      tunnel: w374 -> [w391 w496 w586]
      tunnel: w373 -> [w390 _ _]
      tunnel: w372 -> [w389 w491 _]
      tunnel: w371 -> [w388 w495 w585]
      tunnel: w370 -> [w387 _ _]
      tunnel: w369 -> [w386 w492 _]
      tunnel: [_ _ w587] -> w368
      tunnel: [_ _ w586] -> w367
      tunnel: [_ _ w585] -> w366
      tunnel: [_ _ w584] -> w365
      tunnel: w364 -> [_ w488 _]
      tunnel: [_ w487 _] -> w363
      tunnel: w362 -> [_ w486 _]
      tunnel: [_ w485 _] -> w361
      frame #0 {
        w408 = T5 0 items=["Current", "Voltage"] ("measurement type")
        n193 = call <instrlib>:"niDCPower Configure Current Limit.vi"("current limit"="VG_RSTH_curlim", "channel name"="0", "instrument handle"=w394) -> ("instrument handle out"=w425:refnum<k15>)  [unwired: 7 in, 1 out]
        n194 = call <instrlib>:"niDCPower Configure Current Limit.vi"("current limit"="VTXH_curlim", "channel name"="1", "instrument handle"=w393) -> ("instrument handle out"=w465:refnum<k15>)  [unwired: 7 in, 1 out]
        n195 = call <instrlib>:"niDCPower Configure Current Limit.vi"("current limit"="VGRSTL_curlim", "channel name"="2", "instrument handle"=w392) -> ("instrument handle out"=w466:refnum<k15>)  [unwired: 7 in, 1 out]
        n196 = call <instrlib>:"niDCPower Configure Current Limit.vi"("current limit"="VDDIO_curlim", "channel name"="0", "instrument handle"=w391) -> ("instrument handle out"=w467:refnum<k15>)  [unwired: 7 in, 1 out]
        n197 = call <instrlib>:"niDCPower Configure Current Limit.vi"("current limit"="VDDCL_curlim", "channel name"="1", "instrument handle"=w390) -> ("instrument handle out"=w468:refnum<k15>)  [unwired: 7 in, 1 out]
        n198 = call <instrlib>:"niDCPower Configure Current Limit.vi"("current limit"="VTXL_curlim", "channel name"="2", "instrument handle"=w389) -> ("instrument handle out"=w469:refnum<k15>)  [unwired: 7 in, 1 out]
        n199 = call <instrlib>:"niDCPower Configure Current Limit.vi"("current limit"="VDD13_curlim", "channel name"="0", "instrument handle"=w388) -> ("instrument handle out"=w470:refnum<k15>)  [unwired: 7 in, 1 out]
        n200 = call <instrlib>:"niDCPower Configure Current Limit.vi"("current limit"="VDD33A_curlim", "channel name"="1", "instrument handle"=w387) -> ("instrument handle out"=w438:refnum<k15>)  [unwired: 7 in, 1 out]
        n201 = call <instrlib>:"niDCPower Configure Current Limit.vi"("current limit"="LED_curlim", "channel name"="2", "instrument handle"=w386) -> ("instrument handle out"=w433:refnum<k15>)  [unwired: 7 in, 1 out]
        n202 = call <instrlib>:"niDCPower Configure Current Limit.vi"("current limit"="VDDPIX_curlim", "channel name"="0", "instrument handle"=w383) -> ("instrument handle out"=w418:refnum<k15>)  [unwired: 7 in, 1 out]
        n203 = call <instrlib>:"niDCPower Configure Current Limit.vi"("current limit"="3,3V_LVDS_curlim", "channel name"="1", "instrument handle"=w383) -> ("instrument handle out"=w413:refnum<k15>)  [unwired: 7 in, 1 out]
        n204 = call <instrlib>:"niDCPower Configure Voltage Level.vi"("voltage level"="VG_RSTH, V", "channel name"="0", "instrument handle"=w425) -> ("instrument handle out"=w428:refnum<k15>)  [unwired: 7 in, 1 out]
        n205 = call <instrlib>:"niDCPower Configure Voltage Level.vi"("voltage level"="VTXH, V", "channel name"="1", "instrument handle"=w465) -> ("instrument handle out"=w448:refnum<k15>)  [unwired: 7 in, 1 out]
        n206 = call <instrlib>:"niDCPower Configure Voltage Level.vi"("voltage level"="VGRSTL, V", "channel name"="2", "instrument handle"=w466) -> ("instrument handle out"=w447:refnum<k15>)  [unwired: 7 in, 1 out]
        n207 = call <instrlib>:"niDCPower Configure Voltage Level.vi"("voltage level"="VDDIO, V", "channel name"="0", "instrument handle"=w467) -> ("instrument handle out"=w446:refnum<k15>)  [unwired: 7 in, 1 out]
        n208 = call <instrlib>:"niDCPower Configure Voltage Level.vi"("voltage level"="VDDCL, V", "channel name"="1", "instrument handle"=w468) -> ("instrument handle out"=w445:refnum<k15>)  [unwired: 7 in, 1 out]
        n209 = call <instrlib>:"niDCPower Configure Voltage Level.vi"("voltage level"="VTXL, V", "channel name"="2", "instrument handle"=w469) -> ("instrument handle out"=w444:refnum<k15>)  [unwired: 7 in, 1 out]
        n210 = call <instrlib>:"niDCPower Configure Voltage Level.vi"("voltage level"="VDD13, V", "channel name"="0", "instrument handle"=w470) -> ("instrument handle out"=w443:refnum<k15>)  [unwired: 7 in, 1 out]
        n211 = call <instrlib>:"niDCPower Configure Voltage Level.vi"("voltage level"="VDD33A, V", "channel name"="1", "instrument handle"=w438) -> ("instrument handle out"=w441:refnum<k15>)  [unwired: 7 in, 1 out]
        n212 = call <instrlib>:"niDCPower Configure Voltage Level.vi"("voltage level"="LED, V", "channel name"="2", "instrument handle"=w433) -> ("instrument handle out"=w430:refnum<k15>)  [unwired: 7 in, 1 out]
        n213 = call <instrlib>:"niDCPower Configure Voltage Level.vi"("voltage level"="VDDPIX, V", "channel name"="0", "instrument handle"=w418) -> ("instrument handle out"=w421:refnum<k15>)  [unwired: 7 in, 1 out]
        n214 = call <instrlib>:"niDCPower Configure Voltage Level.vi"("voltage level"="3,3V_LVDS, V", "channel name"="1", "instrument handle"=w413) -> ("instrument handle out"=w410:refnum<k15>)  [unwired: 7 in, 1 out]
        n215 = call <instrlib>:"niDCPower Measure.vi"("measurement type"=w408, "channel name"="0", "instrument handle"=w428) -> ("measurement"=→"VG_RSTH_char" →"VG_RSTH_cur":dbl)  [unwired: 6 in, 2 out]
        n216 = call <instrlib>:"niDCPower Measure.vi"("measurement type"=w408, "channel name"="1", "instrument handle"=w448) -> ("measurement"=→"VTXH_char" →"VTXH_cur":dbl)  [unwired: 6 in, 2 out]
        n217 = call <instrlib>:"niDCPower Measure.vi"("measurement type"=w408, "channel name"="2", "instrument handle"=w447) -> ("measurement"=→"VGRSTL_char" →"VGRSTL_cur":dbl)  [unwired: 6 in, 2 out]
        n218 = call <instrlib>:"niDCPower Measure.vi"("measurement type"=w408, "channel name"="0", "instrument handle"=w446) -> ("measurement"=→"VDDIO_char" →"VDDIO_cur":dbl)  [unwired: 6 in, 2 out]
        n219 = call <instrlib>:"niDCPower Measure.vi"("measurement type"=w408, "channel name"="1", "instrument handle"=w445) -> ("measurement"=→"VDDCL_char" →"VDDCL_cur":dbl)  [unwired: 6 in, 2 out]
        n220 = call <instrlib>:"niDCPower Measure.vi"("measurement type"=w408, "channel name"="2", "instrument handle"=w444) -> ("measurement"=→"VTXL_char" →"VTXL_cur":dbl)  [unwired: 6 in, 2 out]
        n221 = call <instrlib>:"niDCPower Measure.vi"("measurement type"=w408, "channel name"="0", "instrument handle"=w443) -> ("measurement"=→"VDD13_char" →"VDD13_cur":dbl)  [unwired: 6 in, 2 out]
        n222 = call <instrlib>:"niDCPower Measure.vi"("measurement type"=w408, "channel name"="1", "instrument handle"=w441) -> ("measurement"=→"VDD33A_char" →"VDD33A_cur":dbl)  [unwired: 6 in, 2 out]
        n223 = call <instrlib>:"niDCPower Measure.vi"("measurement type"=w408, "channel name"="2", "instrument handle"=w430) -> ("measurement"=→"LED_char":dbl, "instrument handle out"=w396:refnum<k15>)  [unwired: 6 in, 1 out]
        n224 = call <instrlib>:"niDCPower Measure.vi"("measurement type"=w408, "channel name"="0", "instrument handle"=w421) -> ("measurement"=→"VDDPIX_char" →"VDDPIX_cur":dbl)  [unwired: 6 in, 2 out]
        n225 = call <instrlib>:"niDCPower Measure.vi"("measurement type"=w408, "channel name"="1", "instrument handle"=w410) -> ("measurement"=→"3,3V_LVDS_char":dbl)  [unwired: 6 in, 2 out]
        n226 = call <instrlib>:"niDCPower Configure Output Enabled.vi"("output enabled"="LED", "channel name"="2", "instrument handle"=w396) -> ()  [unwired: 7 in, 2 out]
      }
      frame #1 {
        n227 = Greater?(x="Питание", y=w502) -> (0:w500:bool)
        n228 = Less?(x="Питание", y=w502) -> (x < y?=w498:bool)
        n229 = Not(x="Стоп") -> (.not. x?=w499:bool)
        n230 = And(x=w499, y=w500) -> (x .and. y?=w501:bool)
        n231 = Or(x="Стоп", y=w498) -> (x .or. y?=w494:bool)
        n232 = case shown="True" w501 {
          tunnel: w496 -> [_ w549]
          tunnel: w495 -> [_ w548]
          tunnel: w490 -> [_ w547]
          tunnel: w493 -> [_ w546]
          tunnel: w488 -> [w543 w545]
          tunnel: [w543 w544] -> w487
          frame False {
          }
          frame True {
            # "Включение"
            n233 = stacked-sequence {
              tunnel: w549 -> [w550 _ _ _ _ _ w566 _ _ _ _ _ _ _]
              tunnel: w548 -> [_ _ w554 _ w558 _ _ _ _ _ _ _ _ _]
              tunnel: w547 -> [_ _ _ _ _ _ w569 _ _ _ _ _ _ _]
              tunnel: w546 -> [_ _ _ _ _ _ w565 _ _ _ _ _ _ _]
              tunnel: w545 -> [_ _ _ _ _ _ _ _ w573 _ w577 _ _ _]
              tunnel: [_ _ _ _ _ _ _ _ _ _ w576 _ _ _] -> w544
              frame #0 {
                # "VDDIO"
                n234 = call <instrlib>:"niDCPower Configure Output Enabled.vi"("output enabled"=TRUE, "channel name"="0", "instrument handle"=w550) -> ()  [unwired: 7 in, 2 out]
              }
              frame #1 {
                n235 = Wait (ms)(milliseconds to wait=u32 50) -> ()  [unwired: 1 out]
              }
              frame #2 {
                # "VDD13"
                n236 = call <instrlib>:"niDCPower Configure Output Enabled.vi"("output enabled"=TRUE, "channel name"="0", "instrument handle"=w554) -> ()  [unwired: 7 in, 2 out]
              }
              frame #3 {
                n237 = Wait (ms)(milliseconds to wait=u32 50) -> ()  [unwired: 1 out]
              }
              frame #4 {
                # "VDD33А"
                n238 = call <instrlib>:"niDCPower Configure Output Enabled.vi"("output enabled"=TRUE, "channel name"="1", "instrument handle"=w558) -> ()  [unwired: 7 in, 2 out]
              }
              frame #5 {
                n239 = Wait (ms)(milliseconds to wait=u32 50) -> ()  [unwired: 1 out]
              }
              frame #6 {
                n240 = call <instrlib>:"niDCPower Configure Output Enabled.vi"("output enabled"=TRUE, "channel name"="0,1,2", "instrument handle"=w569) -> ()  [unwired: 7 in, 2 out]
                n241 = call <instrlib>:"niDCPower Configure Output Enabled.vi"("output enabled"=TRUE, "channel name"="1,2", "instrument handle"=w566) -> ()  [unwired: 7 in, 2 out]
                n242 = call <instrlib>:"niDCPower Configure Output Enabled.vi"("output enabled"=TRUE, "channel name"="0,1", "instrument handle"=w565) -> ()  [unwired: 7 in, 2 out]
              }
              frame #7 {
                n243 = Wait (ms)(milliseconds to wait=u32 50) -> ()  [unwired: 1 out]
              }
              frame #8 {
                n244 = xnode "Read/Write Control"("FPGA VI Reference In"=w573, "Автомат"=TRUE) -> ()  [unwired: 1 in, 2 out]
              }
              frame #9 {
                n245 = Wait (ms)(milliseconds to wait=u32 1) -> ()  [unwired: 1 out]
              }
              frame #10 {
                n246 = xnode "Read/Write Control"("FPGA VI Reference In"=w577, "SYS_RST_N"=TRUE) -> ("FPGA VI Reference Out"=w576:refnum<k20>)  [unwired: 1 in, 1 out]
              }
              frame #11 {
                n247 = Wait (ms)(milliseconds to wait=u32 1) -> ()  [unwired: 1 out]
              }
              frame #12 {
                # "Прошиваем регистры"
                n248 = local write "W(T)/R(F)"(TRUE ("SPI")) -> ()
                n249 = local write "SPI"(TRUE ("SPI")) -> ()
                n250 = Wait (ms)(milliseconds to wait=u32 10) -> ()  [unwired: 1 out]
              }
              frame #13 {
                n251 = local write "SPI"(FALSE ("SPI")) -> ()
                n252 = local write "НИ"(TRUE ("НИ")) -> ()
              }
            }
          }
        }
        n253 = case shown="True" w494 {
          tunnel: w491 -> [_ w509]
          tunnel: w492 -> [_ w508]
          tunnel: w490 -> [_ w507]
          tunnel: w493 -> [_ w506]
          tunnel: w486 -> [w503 w505]
          tunnel: [w503 w504] -> w485
          frame False {
          }
          frame True {
            # "Выключение"
            n254 = stacked-sequence {
              tunnel: w509 -> [_ _ _ _ w522 _ _ _ _ _ w539 _]
              tunnel: w508 -> [_ _ _ _ _ _ w528 _ w532 _ w538 _]
              tunnel: w507 -> [_ _ _ _ w525 _ _ _ _ _ _ _]
              tunnel: w506 -> [_ _ _ _ w521 _ _ _ _ _ _ _]
              tunnel: w505 -> [w511 _ w516 _ _ _ _ _ _ _ _ _]
              tunnel: [_ _ w514 _ _ _ _ _ _ _ _ _] -> w504
              frame #0 {
                n255 = xnode "Read/Write Control"("FPGA VI Reference In"=w511, "SYS_RST_N"=FALSE) -> ()  [unwired: 1 in, 2 out]
                "НИ" <- FALSE ("НИ")
              }
              frame #1 {
                n256 = Wait (ms)(milliseconds to wait=u32 1) -> ()  [unwired: 1 out]
              }
              frame #2 {
                n257 = xnode "Read/Write Control"("FPGA VI Reference In"=w516, "Автомат"=FALSE) -> ("FPGA VI Reference Out"=w514:refnum<k20>)  [unwired: 1 in, 1 out]
              }
              frame #3 {
                n258 = Wait (ms)(milliseconds to wait=u32 1) -> ()  [unwired: 1 out]
              }
              frame #4 {
                n259 = call <instrlib>:"niDCPower Configure Output Enabled.vi"("output enabled"=FALSE, "channel name"="0,1,2", "instrument handle"=w525) -> ()  [unwired: 7 in, 2 out]
                n260 = call <instrlib>:"niDCPower Configure Output Enabled.vi"("output enabled"=FALSE, "channel name"="1,2", "instrument handle"=w522) -> ()  [unwired: 7 in, 2 out]
                n261 = call <instrlib>:"niDCPower Configure Output Enabled.vi"("output enabled"=FALSE, "channel name"="0,1", "instrument handle"=w521) -> ()  [unwired: 7 in, 2 out]
              }
              frame #5 {
                n262 = Wait (ms)(milliseconds to wait=u32 50) -> ()  [unwired: 1 out]
              }
              frame #6 {
                # "VDD33А"
                n263 = call <instrlib>:"niDCPower Configure Output Enabled.vi"("output enabled"=FALSE, "channel name"="1", "instrument handle"=w528) -> ()  [unwired: 7 in, 2 out]
              }
              frame #7 {
                n264 = Wait (ms)(milliseconds to wait=u32 50) -> ()  [unwired: 1 out]
              }
              frame #8 {
                # "VDD13"
                n265 = call <instrlib>:"niDCPower Configure Output Enabled.vi"("output enabled"=FALSE, "channel name"="0", "instrument handle"=w532) -> ()  [unwired: 7 in, 2 out]
              }
              frame #9 {
                n266 = Wait (ms)(milliseconds to wait=u32 50) -> ()  [unwired: 1 out]
              }
              frame #10 {
                # "VDDIO"
                n267 = call <instrlib>:"niDCPower Configure Output Enabled.vi"("output enabled"=FALSE, "channel name"="0", "instrument handle"=w539) -> ()  [unwired: 7 in, 2 out]
                n268 = call <instrlib>:"niDCPower Configure Output Enabled.vi"("output enabled"=FALSE, "channel name"="2", "instrument handle"=w538) -> ()  [unwired: 7 in, 2 out]
              }
              frame #11 {
                n269 = Wait (ms)(milliseconds to wait=u32 50) -> ()  [unwired: 1 out]
              }
            }
          }
        }
      }
      frame #2 {
        n270 = local read "Стоп"() -> (w588:bool)
      }
    }
    n271 = Wait (ms)(milliseconds to wait=u32 1) -> ()  [unwired: 1 out]
  }
  n272 = while {
    tunnel: w30 -> [w591]
    shift-right: [w595] -> _
    shift-left: FALSE ("Питание") -> [w596]
    tunnel: w31 -> [w593]
    tunnel: [w590] -> w32
    tunnel: [w589] -> w16
    tunnel: w28 -> [_]
    stop <- w592 stop-if-true
    n273 = stacked-sequence {
      tunnel: w596 -> [w599 _ _]
      tunnel: [w598 _ _] -> w595
      tunnel: w593 -> [_ w700 _]
      tunnel: [_ _ w720] -> w592
      tunnel: w591 -> [_ _ w719]
      tunnel: [_ w689 _] -> w590
      tunnel: [_ _ w717] -> w589
      frame #0 {
        n274 = flat-sequence {
          tunnel: w597 -> [w600]
          frame #0 {
            n275 = case shown="True" w600 {
              frame False {
              }
              frame True {
                n276 = Wait (ms)(milliseconds to wait=u32 500) -> ()  [unwired: 1 out]
              }
            }
          }
          frame #1 {
            n277 = local read "VTXH_cur"() -> (w622:dbl)
            n278 = local read "VG_RSTH_cur"() -> (w621:dbl)
            n279 = local read "VGRSTL_cur"() -> (w623:dbl)
            n280 = local read "VDDIO_cur"() -> (w624:dbl)
            n281 = local read "VDDCL_cur"() -> (w615:dbl)
            n282 = local read "VTXL_cur"() -> (w614:dbl)
            n283 = local read "VDD13_cur"() -> (w613:dbl)
            n284 = local read "VDD33A_cur"() -> (w612:dbl)
            n285 = local read "VDDPIX_cur"() -> (w611:dbl)
            n286 = Greater Or Equal?(x=w611, y="VDDPIX_selcur") -> (x >= y?=w602:bool)
            "VDDPIX" <- w602
            n287 = Greater Or Equal?(x=w614, y="VTXL_selcur") -> (x >= y?=w605:bool)
            "VTXL" <- w605
            n288 = Greater Or Equal?(x=w612, y="VDD33A_selcur") -> (x >= y?=w603:bool)
            "VDD33A" <- w603
            n289 = Greater Or Equal?(x=w622, y="VTXH_selcur") -> (x >= y?=w609:bool)
            "VTXH" <- w609
            n290 = Greater Or Equal?(x=w615, y="VDDCL_selcur") -> (x >= y?=w606:bool)
            "VDDCL" <- w606
            n291 = Greater Or Equal?(x=w613, y="VDD13_selcur") -> (x >= y?=w604:bool)
            "VDD13" <- w604
            n292 = Greater Or Equal?(x=w621, y="VG_RSTH_selcur") -> (x >= y?=w610:bool)
            "VG_RSTH" <- w610
            n293 = Greater Or Equal?(x=w623, y="VGRSTL_selcur") -> (x >= y?=w608:bool)
            "VGRSTL" <- w608
            n294 = Greater Or Equal?(x=w624, y="VDDIO_selcur") -> (x >= y?=w607:bool)
            "VDDIO" <- w607
            n295 = case shown="True" w610 {
              frame False {
              }
              frame True {
                n296 = local read "VG_RSTH"() -> (w645:u16)
                n297 = Increment(x=w645) -> (x+1=→"VG_RSTH":u16)
              }
            }
            n298 = case shown="True" w608 {
              frame False {
              }
              frame True {
                n299 = local read "VGRSTL"() -> (w641:u16)
                n300 = Increment(x=w641) -> (x+1=→"VGRSTL":u16)
              }
            }
            n301 = case shown="True" w607 {
              frame False {
              }
              frame True {
                n302 = local read "VDDIO"() -> (w639:u16)
                n303 = Increment(x=w639) -> (x+1=→"VDDIO":u16)
              }
            }
            n304 = case shown="True" w609 {
              frame False {
              }
              frame True {
                n305 = local read "VTXH"() -> (w643:u16)
                n306 = Increment(x=w643) -> (x+1=→"VTXH":u16)
              }
            }
            n307 = case shown="True" w606 {
              frame False {
              }
              frame True {
                n308 = local read "VDDCL"() -> (w637:u16)
                n309 = Increment(x=w637) -> (x+1=→"VDDCL":u16)
              }
            }
            n310 = case shown="True" w605 {
              frame False {
              }
              frame True {
                n311 = local read "VTXL"() -> (w635:u16)
                n312 = Increment(x=w635) -> (x+1=→"VTXL":u16)
              }
            }
            n313 = case shown="True" w604 {
              frame False {
              }
              frame True {
                n314 = local read "VDD13"() -> (w633:u16)
                n315 = Increment(x=w633) -> (x+1=→"VDD13":u16)
              }
            }
            n316 = case shown="True" w603 {
              frame False {
              }
              frame True {
                n317 = local read "VDD33A"() -> (w631:u16)
                n318 = Increment(x=w631) -> (x+1=→"VDD33A":u16)
              }
            }
            n319 = case shown="True" w602 {
              frame False {
              }
              frame True {
                n320 = local read "VDDPIX"() -> (w629:u16)
                n321 = Increment(x=w629) -> (x+1=→"VDDPIX":u16)
              }
            }
          }
        }
        n322 = local read "Питание"() -> (w598:bool)
        n323 = Greater?(x=w598, y=w599) -> (0:w597:bool)
      }
      frame #1 {
        w671 = "\t"
        w687 = i16 0 ("width (-)")
        w688 = i16 3 ("width (-)")
        n324 = local read "VTXH_cur"() -> (w698:dbl)
        n325 = local read "VTXH"() -> (w679:u16)
        n326 = local read "VG_RSTH_cur"() -> (w699:dbl)
        n327 = local read "VGRSTL_cur"() -> (w690:dbl)
        n328 = local read "VDDIO_cur"() -> (w686:dbl)
        n329 = local read "VDDCL_cur"() -> (w685:dbl)
        n330 = local read "VTXL_cur"() -> (w684:dbl)
        n331 = local read "VDD13_cur"() -> (w683:dbl)
        n332 = local read "VDD33A_cur"() -> (w682:dbl)
        n333 = local read "VDDPIX_cur"() -> (w681:dbl)
        n334 = local read "VG_RSTH"() -> (w680:u16)
        n335 = local read "VGRSTL"() -> (w678:u16)
        n336 = local read "VDDIO"() -> (w677:u16)
        n337 = local read "VDDCL"() -> (w676:u16)
        n338 = local read "VTXL"() -> (w675:u16)
        n339 = local read "VDD13"() -> (w674:u16)
        n340 = local read "VDD33A"() -> (w673:u16)
        n341 = local read "VDDPIX"() -> (w672:u16)
        n342 = Get Date/Time In Seconds() -> (seconds since 1Jan1904=w705:timestamp)
        n343 = Format Date/Time String(time format string (%c)="%d %H:%M:%S:%3u", seconds (now)=w705) -> (date/time string=w697:string)  [unwired: 1 in]
        n344 = Number To Fractional String(number=w699, width (-)=w688, precision (6)=w688) -> (F-format string=w696:string)  [unwired: 1 in]
        n345 = Number To Fractional String(number=w698, width (-)=w688, precision (6)=w688) -> (F-format string=w695:string)  [unwired: 1 in]
        n346 = Number To Fractional String(number=w690, width (-)=w688, precision (6)=w688) -> (F-format string=w694:string)  [unwired: 1 in]
        n347 = Number To Fractional String(number=w686, width (-)=w688, precision (6)=w688) -> (F-format string=w693:string)  [unwired: 1 in]
        n348 = Number To Fractional String(number=w685, width (-)=w688, precision (6)=w688) -> (F-format string=w692:string)  [unwired: 1 in]
        n349 = Number To Fractional String(number=w684, width (-)=w688, precision (6)=w688) -> (F-format string=w670:string)  [unwired: 1 in]
        n350 = Number To Fractional String(number=w683, width (-)=w688, precision (6)=w688) -> (F-format string=w669:string)  [unwired: 1 in]
        n351 = Number To Fractional String(number=w682, width (-)=w688, precision (6)=w688) -> (F-format string=w668:string)  [unwired: 1 in]
        n352 = Number To Fractional String(number=w681, width (-)=w688, precision (6)=w688) -> (F-format string=w667:string)  [unwired: 1 in]
        n353 = Number To Fractional String(number=w680, width (-)=w687, precision (6)=w687) -> (F-format string=w666:string)  [unwired: 1 in]
        n354 = Number To Fractional String(number=w679, width (-)=w687, precision (6)=w687) -> (F-format string=w665:string)  [unwired: 1 in]
        n355 = Number To Fractional String(number=w678, width (-)=w687, precision (6)=w687) -> (F-format string=w664:string)  [unwired: 1 in]
        n356 = Number To Fractional String(number=w677, width (-)=w687, precision (6)=w687) -> (F-format string=w663:string)  [unwired: 1 in]
        n357 = Number To Fractional String(number=w676, width (-)=w687, precision (6)=w687) -> (F-format string=w662:string)  [unwired: 1 in]
        n358 = Number To Fractional String(number=w675, width (-)=w687, precision (6)=w687) -> (F-format string=w661:string)  [unwired: 1 in]
        n359 = Number To Fractional String(number=w674, width (-)=w687, precision (6)=w687) -> (F-format string=w660:string)  [unwired: 1 in]
        n360 = Number To Fractional String(number=w673, width (-)=w687, precision (6)=w687) -> (F-format string=w659:string)  [unwired: 1 in]
        n361 = Number To Fractional String(number=w672, width (-)=w687, precision (6)=w687) -> (F-format string=w658:string)  [unwired: 1 in]
        n362 = local read "VG_RSTH"() -> (w655:bool)
        n363 = local read "VDD33A"() -> (w648:bool)
        n364 = local read "VGRSTL"() -> (w653:bool)
        n365 = local read "VDDPIX"() -> (w647:bool)
        n366 = local read "VDDCL"() -> (w651:bool)
        n367 = local read "VDDIO"() -> (w652:bool)
        n368 = local read "VDD13"() -> (w649:bool)
        n369 = local read "VTXH"() -> (w654:bool)
        n370 = local read "VTXL"() -> (w650:bool)
        n371 = Compound Arithmetic op=OR(w655, w654, w653, w652, w651, w650, w649, w648, w647) -> (w691:bool)
        n372 = Select(t="!!!", s=w691, f="") -> (s? t:f=w657:string)
        n373 = Concatenate Strings(w697, w671, w696, w671, w695, w671, w694, w671, w693, w671, w692, w671, w670, w671, w669, w671, w668, w671, w667, w671, w666, w671, w665, w671, w664, w671, w663, w671, w662, w671, w661, w671, w660, w671, w659, w671, w658, w671, w657, "\r\n") -> (w701:string)
        n374 = Format Into String(initial string=w700, w701) -> (resulting string=w689:refnum<file>)  [unwired: 2 in, 1 out]
      }
      frame #2 {
        n375 = local read "VG_RSTH"() -> (w715:bool)
        n376 = local read "Питание"() -> (w718:bool)
        n377 = local read "VDD33A"() -> (w708:bool)
        n378 = local read "VGRSTL"() -> (w713:bool)
        n379 = local read "VDDPIX"() -> (w707:bool)
        n380 = local read "VDDCL"() -> (w711:bool)
        n381 = local read "VDDIO"() -> (w712:bool)
        n382 = local read "VDD13"() -> (w709:bool)
        n383 = local read "VTXH"() -> (w714:bool)
        n384 = local read "VTXL"() -> (w710:bool)
        n385 = Compound Arithmetic op=OR(w715, w714, w713, w712, w711, w710, w709, w708, w707, "SIM_SEL") -> (w716:bool)
        "SEL" <- w716
        n386 = case shown="True" w716 {
          tunnel: [w722 w730] -> w720
          tunnel: w719 -> [w721 w729]
          tunnel: w718 -> [_ w726]
          tunnel: [w721 w725] -> w717
          frame False {
            n387 = local read "Стоп"() -> (w722:bool)
          }
          frame True {
            n388 = flat-sequence {
              tunnel: w729 -> [w734]
              tunnel: [w732] -> w727
              tunnel: w726 -> [w732]
              tunnel: [w731] -> w723
              tunnel: [w737] -> w728
              tunnel: w727 -> [w737]
              tunnel: [w736] -> w724
              tunnel: w723 -> [w736]
              tunnel: [w741] -> w730
              tunnel: w728 -> [w740]
              tunnel: [w739] -> w725
              tunnel: w724 -> [w739]
              frame #0 {
                n389 = local write "Питание"(FALSE ("Питание")) -> ()
                n390 = xnode "Read/Write Control"("FPGA VI Reference In"=w734, "Автомат"=FALSE ("Линейки")) -> ("FPGA VI Reference Out"=w731:refnum<k20>)  [unwired: 1 in, 1 out]
              }
              frame #1 {
                n391 = Wait (ms)(milliseconds to wait="SEL_Time, ms") -> ()  [unwired: 1 out]
              }
              frame #2 {
                n392 = local write "Питание"(w740) -> ()
                n393 = local read "Стоп"() -> (w741:bool)
              }
            }
          }
        }
      }
    }
    n394 = Wait (ms)(milliseconds to wait="Период опроса, мс") -> ()  [unwired: 1 out]
  }
  n395 = while {
    tunnel: w13 -> [w745]
    tunnel: [w743] -> w8
    stop <- w744 stop-if-true
    n396 = feedback #2() -> (w747:bool)  [unwired: 1 in]
    n397 = feedback-in #2("SPI") -> ()
    n398 = Greater?(x="SPI", y=w747) -> (0:w746:bool)
    n399 = case shown="True" w746 {
      selector: w746 -> [_ w753]
      tunnel: w745 -> [w748 w754]
      tunnel: [w750 w752] -> w744
      tunnel: [w748 w751] -> w743
      frame False {
        n400 = Wait (ms)(milliseconds to wait=u32 1) -> ()  [unwired: 1 out]
        n401 = local read "Стоп"() -> (w750:bool)
      }
      frame True {
        n402 = stacked-sequence {
          seq-local: [_ _ _ _ _ _ _ w776 _] -> [_ _ _ _ _ _ _ _ w783]
          tunnel: w754 -> [w765 _ w768 _ w772 _ w775 w779 w784]
          tunnel: w753 -> [_ _ _ _ _ _ _ _ _]
          tunnel: [_ _ _ _ _ _ _ _ w785] -> w752
          tunnel: [w759 _ _ _ _ _ _ _ _] -> w751
          frame #0 {
            n403 = local write "Прошили"(FALSE ("Прошили")) -> ()
            n404 = xnode "Read/Write Control"("FPGA VI Reference In"=w765, "W(T)/R(F)"="W(T)/R(F)", "Адрес"="Адрес", "Кол-во"="Кол-во", "12 2"="12", "FR"="FR", "19"=u8 18, "20"=u8 19, "2372000"=u32 2372000) -> ("FPGA VI Reference Out"=w759:refnum<k20>)  [unwired: 1 in, 1 out]
          }
          frame #1 {
            n405 = Wait (ms)(milliseconds to wait=u32 1) -> ()  [unwired: 1 out]
          }
          frame #2 {
            n406 = xnode "Read/Write Control"("FPGA VI Reference In"=w768, "SPI"=TRUE) -> ()  [unwired: 1 in, 2 out]
          }
          frame #3 {
            n407 = Wait (ms)(milliseconds to wait=u32 1) -> ()  [unwired: 1 out]
          }
          frame #4 {
            n408 = xnode "Read/Write Control"("FPGA VI Reference In"=w772, "SPI"=FALSE, "Upd_RD"=TRUE) -> ()  [unwired: 1 in, 2 out]
          }
          frame #5 {
            n409 = Wait (ms)(milliseconds to wait=u32 1) -> ()  [unwired: 1 out]
          }
          frame #6 {
            n410 = xnode "Read/Write Control"("FPGA VI Reference In"=w775, "Upd_RD"=FALSE) -> ()  [unwired: 1 in, 2 out]
          }
          frame #7 {
            n411 = xnode "Invoke Method"("FPGA VI Reference In"=w779, "Number of Elements"=u32 0, "Timeout (ms)"=0) -> ("Elements Remaining"=w776:u32)  [unwired: 1 in, 3 out]
            "FIFO_READ" <- w776
          }
          frame #8 {
            n412 = xnode "Invoke Method"("FPGA VI Reference In"=w784, "Number of Elements"=w783, "Timeout (ms)"=0) -> ("Data"=→"READ":u8[])  [unwired: 1 in, 3 out]
            n413 = local read "Стоп"() -> (w785:bool)
            "Прошили" <- TRUE ("Прошили")
          }
        }
      }
    }
  }
  n414 = call <instrlib>:"niDCPower Close.vi"("instrument handle"=w24) -> ()  [unwired: 10 in, 1 out]
  n415 = call <instrlib>:"niDCPower Close.vi"("instrument handle"=w23) -> ()  [unwired: 10 in, 1 out]
  n416 = call <instrlib>:"niDCPower Close.vi"("instrument handle"=w22) -> ()  [unwired: 10 in, 1 out]
  n417 = call <instrlib>:"niDCPower Close.vi"("instrument handle"=w25) -> ()  [unwired: 10 in, 1 out]
  n418 = Close File(refnum=w32) -> ()  [unwired: 1 in, 2 out]
  n419 = flat-sequence {
    tunnel: w16 -> [_]
    tunnel: w11 -> [w787]
    tunnel: w9 -> [_]
    tunnel: w8 -> [_]
    tunnel: w7 -> [_]
    tunnel: w2 -> [_]
    frame #0 {
      n420 = xnode "Read/Write Control"("FPGA VI Reference In"=w787, "Стоп"=TRUE) -> ("FPGA VI Reference Out"=w788:refnum<k20>)  [unwired: 1 in, 1 out]
      n421 = xnode "Close FPGA VI Reference"("FPGA VI Reference In"=w788) -> ()  [unwired: 1 in, 1 out]
    }
  }
  n422 = Close File(refnum=w14) -> ()  [unwired: 1 in, 2 out]
